vi "Gating Function.vi"() -> ()   [LabVIEW 2026]
panel:
  in  "Loop Rate (ms)":u32=10
  out "Loop Iteration":i32
  out "Outputs":bool[](array[boolean])
  in  "Stop":bool
  in  "Simulated Inputs":bool[](array[boolean])
  in  "Gate Switch":bool
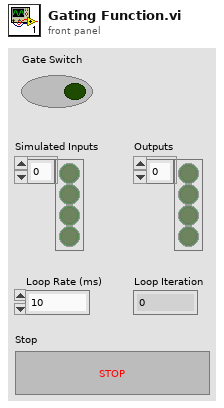
[diagram p1: front panel]
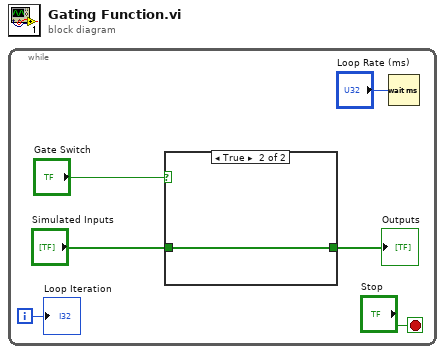
[diagram p0: block diagram]
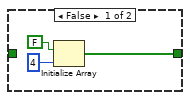
[diagram p2: hidden frame]
diagram:
  n1 = while {
    i -> [w3]
    stop <- "Stop" stop-if-true
    n2 = case shown="True" "Gate Switch" {
      tunnel: [w7 w10] -> w2
      tunnel: "Simulated Inputs" -> [_ w10]
      frame False {
        n3 = Initialize Array(FALSE, 4 ("dimension size")) -> (w7:bool[])
      }
      frame True {
      }
    }
    "Outputs" <- w2
    n4 = Wait (ms)(milliseconds to wait="Loop Rate (ms)") -> ()  [unwired: 1 out]
    "Loop Iteration" <- w3
  }
